vi "PicoScope5000aExampleAdvancedTriggerV2.vi"() -> ()   [LabVIEW 2010]
doc: "This example demonstrates how to use the PicoScope Labview library to collect data using Advanced triggers in block mode."
uses:
  shared/PicoBuffers.ctl
  <vilib>/Waveform/DWDTOps.llb/DWDT Analog to Digital.vi
  PicoScope5000aLib/PicoScope5000aDigitalChannelSettings.ctl
  PicoScope5000aLib/PicoScope5000aAnalogChannelSettings.ctl
  shared/Buffer and Transfer Settings.ctl
  shared/Acquisition Settings.ctl
panel:
  in  "Write to TDMS":bool
  in  "roundFaster":bool=TRUE
  in  "timeIntervalRequested":dbl min=0.0 format="%#6_6p"
  in  "Pulse Width Qualifier Settings":T1={"Direction"=2, "Lower Limit"=0, "Upper Limit"=0, "Pulse Width Type"=0} {"Pulse Width Type" items=["None", "Less Than", "Greater Than", "In Range", "Out of Range"]; "Direction" items=["Rising"=2, "Falling"=3, "Rising Lower"=7, "Above"=0, "Below"=1, "Rising or Falling"=4, "Falling Lower"=8, "Below Lower"=6, "Above Lower"=5]}
  in  "Trigger Conditions":T2={"Channel A"=1, "Channel B"=0, "Channel C"=0, "Channel D"=0, "Ext"=0, "Aux"=0, "PWQ"=0, "Digital Port 0"=0, "Digital Port 1"=0, "Condition Logic"=0} {"Digital Port 1" items=["Don't Care", "True", "False"]; "Digital Port 0" items=["Don't Care", "True", "False"]; "PWQ" items=["Don't Care", "True", "False"]; "Aux" items=["Don't Care", "True", "False"]; "Ext" items=["Don't Care", "True", "False"]; "Channel D" items=["Don't Care", "True", "False"]; "Channel C" items=["Don't Care", "True", "False"]; "Channel B" items=["Don't Care", "True", "False"]; "Channel A" items=["Don't Care", "True", "False"]; "Condition Logic" items=["AND", "OR", "XOR"]}
  in  "Pulse Width Qualifier Conditions":T3 {"Condition Logic" items=["AND", "OR", "XOR"]}
  in  "Digital Port  0":T4 {"Direction Channel 7" items=["Don't Care", "Low", "High", "Rising", "Falling"]; "Direction Channel 6" items=["Don't Care", "Low", "High", "Rising", "Falling"]; "Direction Channel 5" items=["Don't Care", "Low", "High", "Rising", "Falling"]; "Direction Channel 4" items=["Don't Care", "Low", "High", "Rising", "Falling"]; "Direction Channel 3" items=["Don't Care", "Low", "High", "Rising", "Falling"]; "Direction Channel 2" items=["Don't Care", "Low", "High", "Rising", "Falling"]; "Direction Channel 1" items=["Don't Care", "Low", "High", "Rising", "Falling"]; "Direction Channel 0" items=["Don't Care", "Low", "High", "Rising", "Falling"]}
  in  "Channel A Trigger Properties":T5={"thresholdUpper"=0, "thresholdUpperHysteresis"=0, "thresholdLower"=0, "thresholdLowerHysteresis"=0, "Threshold Mode"=0, "Direction"=2, "Available"=TRUE} {"Direction" items=["Above / Inside", "Below / Outside", "Rising / Enter", "Falling / Exit", "Rising or Falling / Enter or Exit", "Above Lower", "Below Lower", "Rising Lower", "Falling Lower", "Positive Runt", "Negative Runt"]; "Threshold Mode" items=["Level", "Window"]}
  out "overflow":i16 format="%010b"
  in  "Apply Settings":bool
  in  "Port 0 Settings":T6={"Enabled"=FALSE, "Logic Level"=9830} {"Logic Level" items=["1.5V TTL"=9830, "2.5V CMOS"=16383]}
  in  "Channel A Settings":T7={"Enabled"=TRUE, "Coupling"=1, "Range"=6, "Analogue Offset"=0.0, "Bandwidth Limit"=0} {"Bandwidth Limit" items=["Full", "20MHz"]; "Range" items=["10 mV", "20 mV", "50 mV", "100 mV", "200 mV", "500 mV", "1 V", "2 V", "5 V", "10 V", "20 V"]; "Coupling" items=["AC", "DC"]}
  out "USB 3.0 device on non-USB 3.0 Port":bool=TRUE
  out "USB Powered":bool=TRUE
  out "Device Info":T8={"Driver Version"="2.1.104.3324", "USB Version"="2.0", "Hardware"="1", "Variant"="5244A", "Batch and Serial"="CQ178/007", "Cal Date"="11Jun13", "Kernel Version"="1.0", "Digital HW Version"="1", "Analogue HW Version"="1", "MSO"=FALSE, "Number of channels"=2}
  out "error out":errorcluster
  in  "Data file":path=path "PicoScope5000aExampleBlock Data"
  in  "Buffer and Transfer Settings":T9={"startIndex"=0, "Samples"=5000000, "Down Sample Ratio"=1, "Down-Sample Mode"=0} {"Down-Sample Mode" items=["RAW none"=2147483648, "None"=0, "Aggregate"=1, "Decimate"=2, "Average"=4]; "Down Sample Ratio" step=1; "Samples" format="%_6p"}
  in  "Acquisition Settings":T10={"preTriggerSamples"=0, "postTriggerSamples"=5000000, "timebase"=0} {"postTriggerSamples" format="%_6p"; "preTriggerSamples" format="%_6p"}
  out "Properties Panel":T11 {"Max Total Capture Time Available (sec)" format="%.3p"; "Sample Frequency" format="%.6p"; "Sample Rate" format="%.3p"; "Max Samples Available" format="%_6p"; "Total Capture Time (sec)" format="%.3p"}
  out "Port 0":digitalwaveform(graph)={"t0"=timestamp(0 s since 1904-01-01), "dt"=8e-09, "Y"={"transitions"=[], "data"=[]}}
  in  "stop":bool
  out "Analog Channels":cluster{i32, sgl, "Data":dbl[]}[](graph)
  in  "Resolution":u32(ring) items=["8-bit"=0, "12-bit"=1, "14-bit"=2, "15-bit"=3, "16-bit"=4, "10-bit"=10]
  in  "Serial Number":string
  in  "Use Serial Number":bool
  in  "error in (no error)":errorcluster
  # "Bit 0 = ChA"
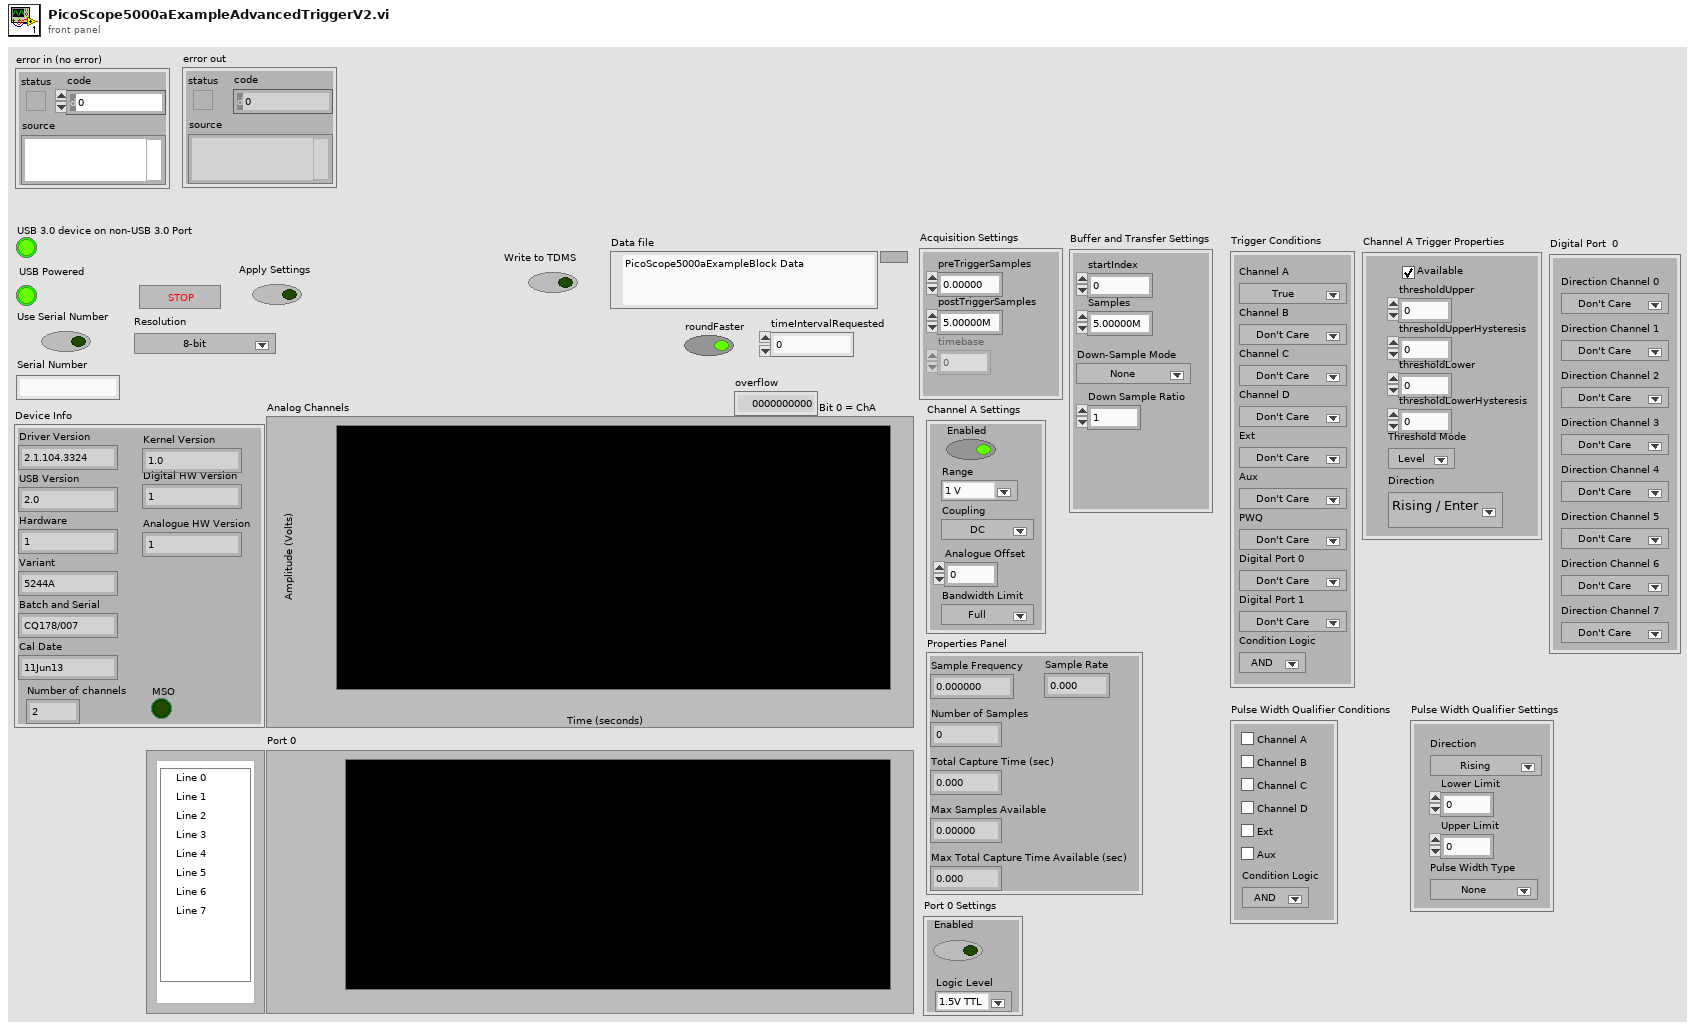
[diagram p1: front panel]
types:
  T1 = cluster{"Direction":u32, "Lower Limit":u32, "Upper Limit":u32, "Pulse Width Type":u32}
  T2 = cluster{"Channel A":u16, "Channel B":u16, "Channel C":u16, "Channel D":u16, "Ext":u16, "Aux":u16, "PWQ":u16, "Digital Port 0":u16, "Digital Port 1":u16, "Condition Logic":u16}
  T3 = cluster{"Channel A":bool, "Channel B":bool, "Channel C":bool, "Channel D":bool, "Aux":bool, "Condition Logic":u16, "Ext":bool}
  T4 = cluster{"Direction Channel 0":u16, "Direction Channel 1":u16, "Direction Channel 2":u16, "Direction Channel 3":u16, "Direction Channel 4":u16, "Direction Channel 5":u16, "Direction Channel 6":u16, "Direction Channel 7":u16}
  T5 = cluster{"thresholdUpper":i16, "thresholdUpperHysteresis":u16, "thresholdLower":i16, "thresholdLowerHysteresis":u16, "Threshold Mode":i32, "Direction":i32, "Available":bool}
  T6 = typedef "PicoScope5000aDigitalChannelSettings.ctl" = cluster{"Enabled":bool, "Logic Level":i16}
  T7 = typedef "PicoScope5000aAnalogChannelSettings.ctl" = cluster{"Enabled":bool, "Coupling":i16, "Range":u16, "Analogue Offset":sgl, "Bandwidth Limit":u32}
  T8 = cluster{"Driver Version":string, "USB Version":string, "Hardware":string, "Variant":string, "Batch and Serial":string, "Cal Date":string, "Kernel Version":string, "Digital HW Version":string, "Analogue HW Version":string, "MSO":bool, "Number of channels":i16}
  T9 = typedef "Buffer and Transfer Settings.ctl" = cluster{"startIndex":u64, "Samples":u64, "Down Sample Ratio":u64, "Down-Sample Mode":u32}
  T10 = typedef "Acquisition Settings.ctl" = cluster{"preTriggerSamples":u64, "postTriggerSamples":u64, "timebase":u32}
  T11 = cluster{"Sample Frequency":dbl, "Sample Rate":dbl, "Max Samples Available":u64, "Number of Samples":u64, "Total Capture Time (sec) ":dbl, "Max Total Capture Time Available (sec)":dbl}
  T12 = typedef "PicoBuffers.ctl" = cluster{"Max Buffer Pointers":u64[][][], "Min Buffer Pointers":u64[][][], "StreamingDataInfo":cluster{"Channel":u32, "Down-Sample Mode":u32, "PICO_DATA_TYPE":enum32{"PICO_INT8_T", "PICO_INT16_T", "PICO_INT32_T", "PICO_UINT32_T", "PICO_INT64_T", ""}, "Samples":i32, "bufferIndex":u64, "startIndex":i32, "overflow":i16}[][]}
  T13 = enum16{"open", "open or create", "create or replace", "create", "open (read-only)"}
  T14 = cluster{"Sample Frequency":sgl, "Sample Rate":sgl, "Max Samples Available":i32, "Number of Samples":u32, "Total Capture Time (sec) ":sgl, "Max Total Capture Time Available (sec)":sgl}
  T15 = cluster{"Channel A Buffer":i16[], "Channel B Buffer":i16[], "Channel C Buffer":i16[], "Channel D Buffer":i16[], "Channel E Buffer":i16[], "Channel F Buffer":i16[], "Channel G Buffer":i16[], "Channel H Buffer":i16[], "Port 0 Buffer":i16[], "Port 1 Buffer":i16[]}[]
  T16 = cluster{"Channel A Buffer":i16[], "Channel B Buffer":i16[], "Channel C Buffer":i16[], "Channel D Buffer":i16[], "Channel E Buffer":i16[], "Channel F Buffer":i16[], "Channel G Buffer":i16[], "Channel H Buffer":i16[], "Port 0 Buffer":i16[], "Port 1 Buffer":i16[]}
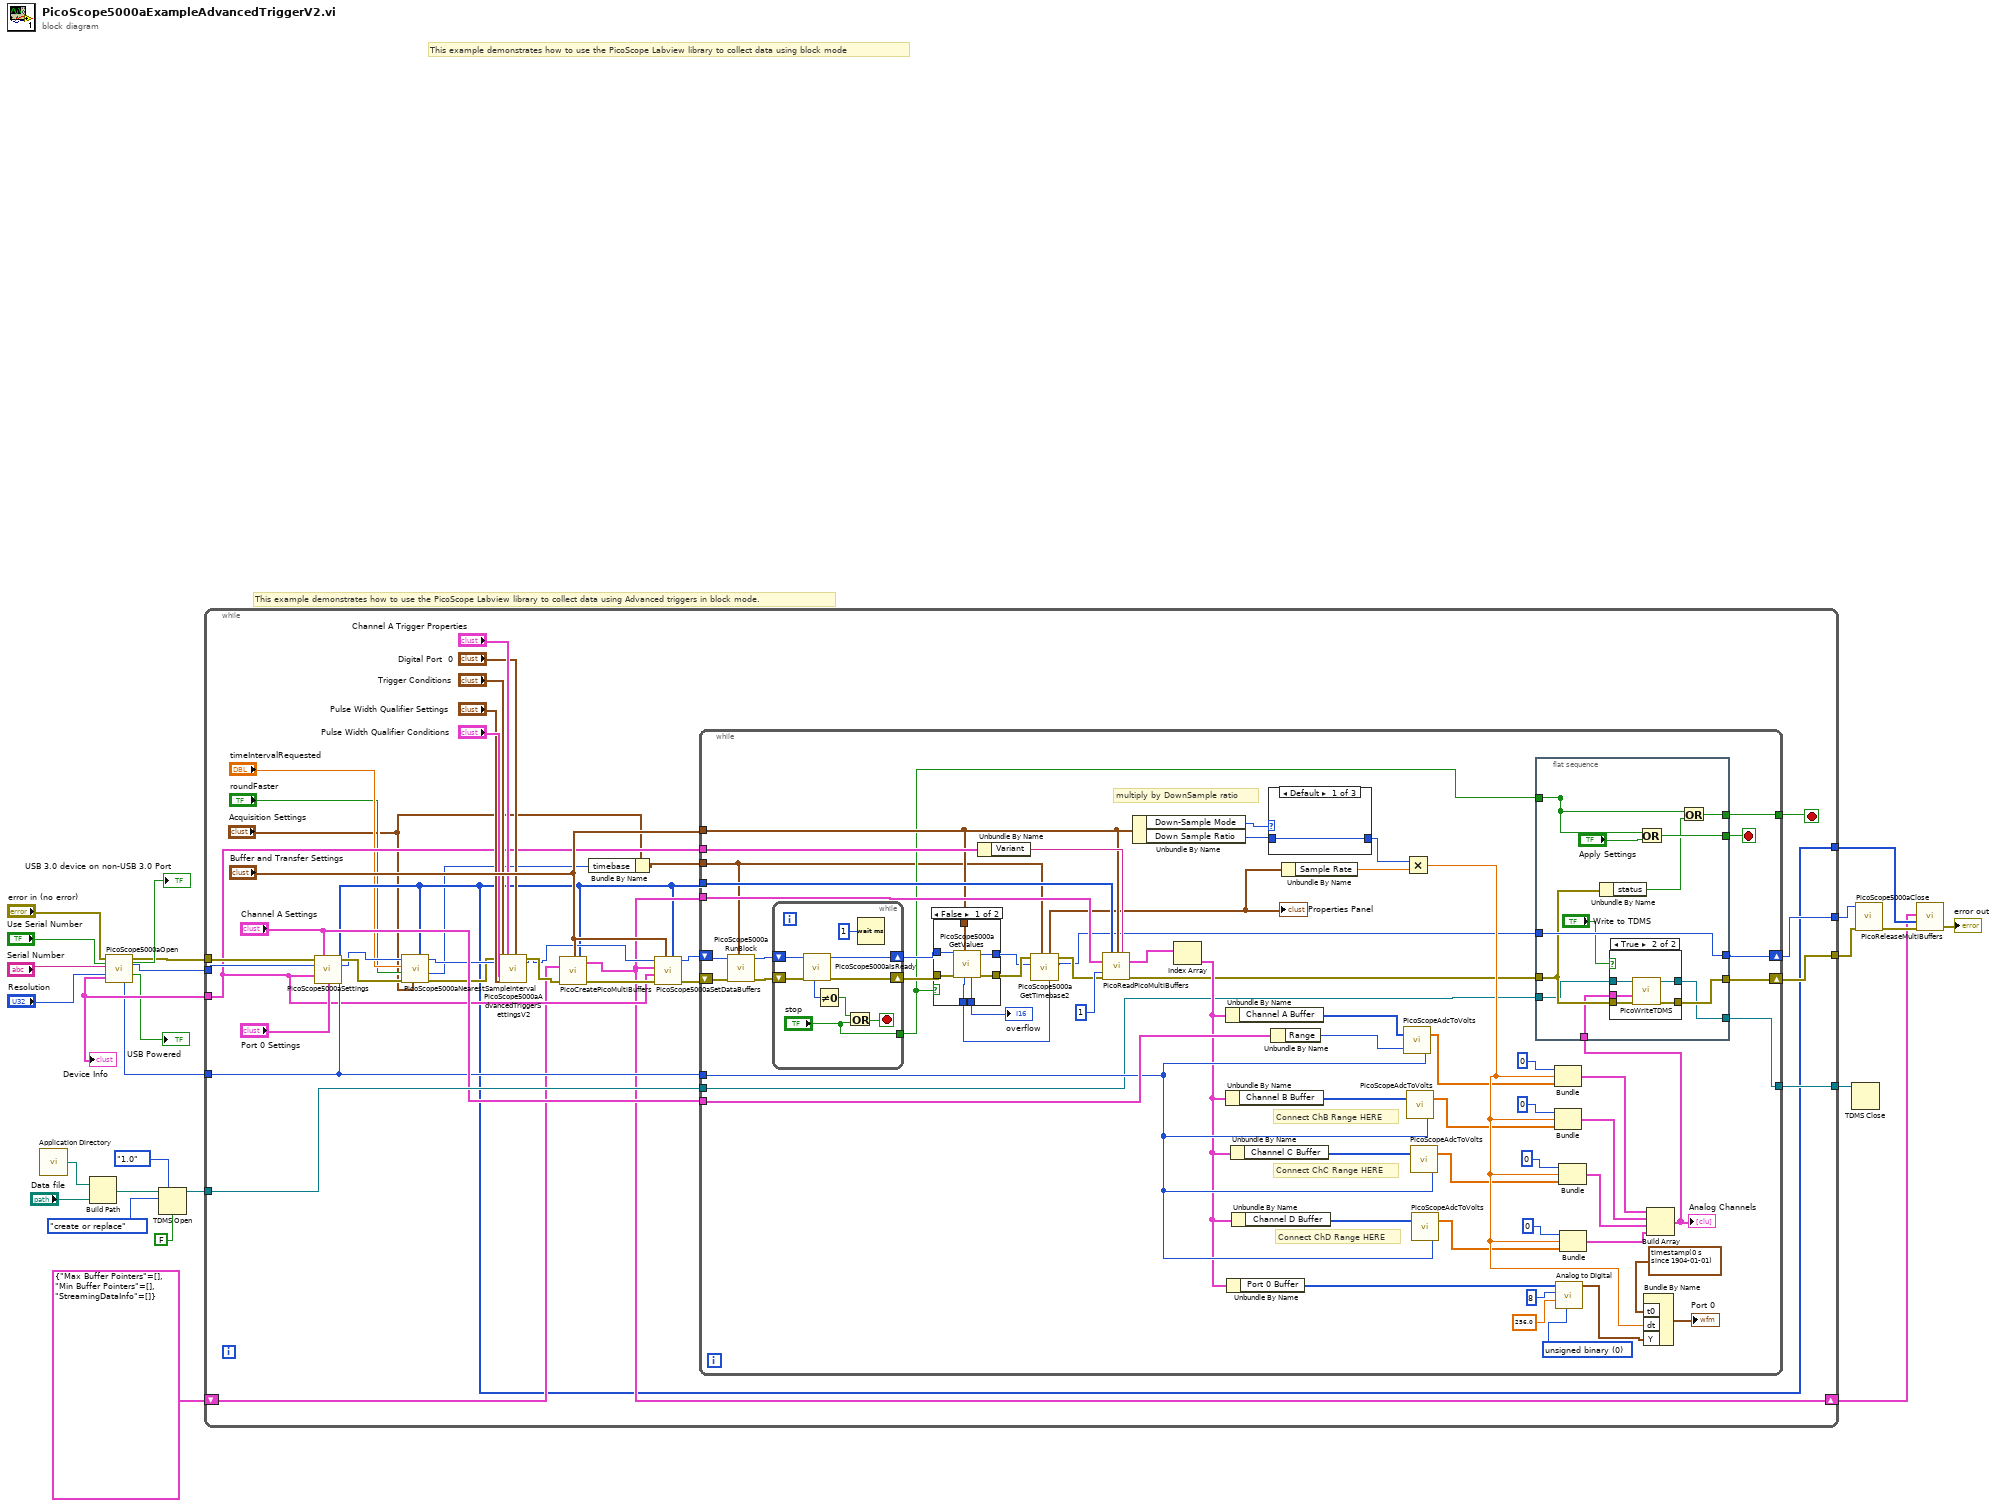
[diagram p0: block diagram]
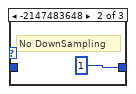
[diagram p4: hidden frame]
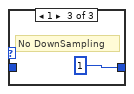
[diagram p5: hidden frame]
diagram:
  # "This example demonstrates how to use the PicoScope Labview library to collect data using Advanced triggers in block mode."
  # "This example demonstrates how to use the PicoScope Labview library to collect data using block mode"
  n1 = call <vilib>:"Application Directory.vi"() -> ("Application Directory"=w18:path)
  n2 = Build Path(base path=w18, name or relative path="Data file") -> (appended path=w19:path)
  n3 = call "PicoScope5000aOpen.vi"("error in (no error)"="error in (no error)", "Serial Number"="Serial Number", "Use Serial Number"="Use Serial Number", "Resolution"="Resolution") -> ("USB 3.0 device on non-USB 3.0 Port"=→"USB 3.0 device on non-USB 3.0 Port":bool, "error out"=w6:errorcluster, "handle"=w25:i16, "USB Powered"=→"USB Powered":bool, "Device Info"=w10:T8, "Max ADC value"=w9:i16)  [unwired: 6 in]
  "Device Info" <- w10
  n4 = TDMS Open(6:FALSE ("disable buffering? (T)"), 7:enum16{"1.0", "2.0"}."1.0" ("file format version (2.0)"), 10:T13."create or replace" ("operation (0:open)"), 11:w19) -> (3:w16:refnum<k34>)  [unwired: 2 in, 1 out]
  n5 = while {
    tunnel: w25 -> [w57]
    tunnel: w9 -> [w53]
    tunnel: [w31] -> w24
    tunnel: [w51] -> w17
    tunnel: w16 -> [w58]
    tunnel: w10 -> [w38]
    tunnel: w6 -> [w56]
    tunnel: [w52] -> w4
    tunnel: [w49] -> w5
    shift-right: [w36] -> w1
    shift-left: T12 {"Max Buffer Pointers"=[], "Min Buffer Pointers"=[], "StreamingDataInfo"=[]} ("Data Pointers") -> [w37]
    stop <- w50 stop-if-true
    n6 = call "PicoScope5000aSettings.vi"("error in"=w56, "Channel A Settings"="Channel A Settings", "Port 0 Settings"="Port 0 Settings", "handle in"=w57, "Device Info"=w38, "Max ADC value"=w53) -> ("error out"=w35:errorcluster, "handle out"=w34:i16, "enabled array"=w31:i16[])  [unwired: 7 in]
    n7 = call "PicoScope5000aNearestSampleInterval.vi"("Enabled array"=w31, "Acquisition Settings"="Acquisition Settings", "error in (no error)"=w35, "roundFaster"="roundFaster", "timeIntervalRequested"="timeIntervalRequested", "handle in"=w34) -> ("error out"=w32:errorcluster, "timebase"=w27:u32, "handle out"=w33:i16)  [unwired: 2 in, 1 out]
    n8 = call "PicoScope5000aAdvancedTriggerSettingsV2.vi"("error in"=w32, "handle in"=w33, "Trigger Conditions"="Trigger Conditions", "Channel A Trigger Properties"="Channel A Trigger Properties", "Digital Port  0"="Digital Port  0", "Pulse Width Qualifier Conditions"="Pulse Width Qualifier Conditions", "Pulse Width Qualifier Settings"="Pulse Width Qualifier Settings") -> ("error out"=w45:errorcluster, "handle out"=w44:i16)  [unwired: 11 in]
    n9 = call "PicoCreatePicoMultiBuffers.vi"("Buffer and Transfer Settings"="Buffer and Transfer Settings", "enabled array"=w31, "Data Pointers In"=w37, "error in (no error)"=w45) -> ("Data Pointers"=w36:T12, "error out"=w59:errorcluster)  [unwired: 10 in]
    n10 = Bundle By Name(cluster="Acquisition Settings", "timebase"=w27) -> (w28:T10)
    n11 = call "PicoScope5000aSetDataBuffers.vi"("enabled array"=w31, "Buffer and Transfer Settings"="Buffer and Transfer Settings", "error in (no error)"=w59, "Device Info"=w38, "Data Pointers In"=w36, "handle in"=w44) -> ("error out"=w48:errorcluster, "handle out"=w47:i16)  [unwired: 4 in]
    n12 = while {
      tunnel: w36 -> [w121]
      tunnel: "Buffer and Transfer Settings" -> [w72]
      tunnel: w31 -> [w113]
      tunnel: "Channel A Settings" -> [w112]
      tunnel: w28 -> [w63]
      tunnel: w53 -> [w111]
      tunnel: w38 -> [w108]
      tunnel: [w79] -> w50
      shift-right: [w81] -> w52
      shift-left: w48 -> [w73]
      shift-right: [w77] -> w49
      shift-left: w47 -> [w74]
      tunnel: w58 -> [w62]
      tunnel: [w60] -> w51
      stop <- w78 stop-if-true
      w98 = u16 0 items=["unsigned binary", "offset binary", "2's complement"] ("data format (offset binary)")
      # "Connect ChB Range HERE"
      # "Connect ChD Range HERE"
      # "Connect ChC Range HERE"
      # "multiply by DownSample ratio"
      n13 = call "PicoScope5000aRunBlock.vi"("Acquisition Settings"=w63, "error in (no error)"=w73, "handle in"=w74) -> ("error out"=w115:errorcluster, "handle out"=w114:i16)  [unwired: 5 in, 2 out]
      n14 = while {
        shift-right: [w157] -> w75
        shift-left: w115 -> [w158]
        shift-right: [w156] -> w76
        shift-left: w114 -> [w155]
        tunnel: ["stop"] -> w71
        stop <- w152 stop-if-true
        n15 = call "PicoScope5000aIsReady.vi"("error in (no error)"=w158, "handle in"=w155) -> ("error out"=w157:errorcluster, "handle out"=w156:i16, "ready"=w154:i16)  [unwired: 7 in]
        n16 = Not Equal To 0?(x=w154) -> (x != 0?=w153:bool)
        n17 = Or(x=w153, y="stop") -> (x .or. y?=w152:bool)
        n18 = Wait (ms)(milliseconds to wait=u32 1) -> ()  [unwired: 1 out]
      }
      n19 = case shown="False" w71 {
        tunnel: w75 -> [w128 w129]
        tunnel: w76 -> [w127 w130]
        tunnel: [w126 w130] -> w68
        tunnel: [w125 w129] -> w69
        tunnel: w72 -> [w124 _]
        tunnel: [w123 _] -> w70
        tunnel: [w122 _] -> w65
        frame False {
          n20 = call "PicoScope5000aGetValues.vi"("Buffer and Transfer Settings"=w124, "error in (no error)"=w128, "handle in"=w127) -> ("error out"=w125:errorcluster, "handle out"=w126:i16, "overflow"=w123:i16, "noOfSamples"=w122:u64)  [unwired: 5 in]
        }
        frame True {
        }
      }
      "overflow" <- w70
      n21 = Unbundle By Name(w108) -> ("Variant"=w109:string)
      n22 = call "PicoScope5000aGetTimebase2.vi"("Number of Samples"=w65, "Acquisition Settings"=w63, "handle in"=w68, "error in (no error)"=w69) -> ("handle out"=w66:i16, "error out"=w67:errorcluster, "Properties Panel"=w64:T14)  [unwired: 5 in]
      "Properties Panel" <- w64
      n23 = call "PicoReadPicoMultiBuffers.vi"("enabled array"=w113, "Buffer and Transfer Settings"=w72, "Variant"=w109, "Data Pointers"=w121, "No of Buffers"=1, "error in (no error)"=w67) -> ("MultiBuffers (Max or non-aggregated)"=w120:T15, "error out"=w80:errorcluster)  [unwired: 7 in, 1 out]
      n24 = Unbundle By Name(w72) -> ("Down-Sample Mode"=w118:u32, "Down Sample Ratio"=w119:u64)
      n25 = Index Array(array=w120) -> (element=w82:T16)  [unwired: 1 in]
      n26 = Unbundle By Name(w82) -> ("Channel A Buffer"=w91:i16[])
      n27 = Unbundle By Name(w82) -> ("Channel B Buffer"=w103:i16[])
      n28 = Unbundle By Name(w82) -> ("Port 0 Buffer"=w96:i16[])
      n29 = Unbundle By Name(w82) -> ("Channel C Buffer"=w89:i16[])
      n30 = Unbundle By Name(w82) -> ("Channel D Buffer"=w85:i16[])
      n31 = case shown="Default" w118 {
        tunnel: [w159 u64 1 ("Down Sample Ratio") u64 1 ("Down Sample Ratio")] -> w116
        tunnel: w119 -> [w159 _ _]
        frame Default {
        }
        frame -2147483648 {
          # "No DownSampling"
        }
        frame 1 {
          # "No DownSampling"
        }
      }
      n32 = Unbundle By Name(w112) -> ("Range"=w105:u16)
      n33 = Unbundle By Name(w64) -> ("Sample Rate"=w110:sgl)
      n34 = call "PicoScopeAdcToVolts.vi"("Max_adc"=w111, "Range Index"=w105, "Data"=w91) -> ("Data"=w92:dbl[])
      n35 = Multiply(x=w116, y=w110) -> (x*y=w117:sgl)
      n36 = call "PicoScopeAdcToVolts.vi"("Max_adc"=w111, "Data"=w103) -> ("Data"=w102:dbl[])  [unwired: 1 in]
      n37 = call "PicoScopeAdcToVolts.vi"("Max_adc"=w111, "Data"=w89) -> ("Data"=w88:dbl[])  [unwired: 1 in]
      n38 = call "PicoScopeAdcToVolts.vi"("Max_adc"=w111, "Data"=w85) -> ("Data"=w84:dbl[])  [unwired: 1 in]
      n39 = flat-sequence {
        tunnel: [w142] -> w78
        tunnel: [w137] -> _
        tunnel: [w139] -> w79
        tunnel: w66 -> [w138]
        tunnel: [w138] -> w77
        tunnel: w80 -> [w135]
        tunnel: [w136] -> w81
        tunnel: w71 -> [w137]
        tunnel: w62 -> [w134]
        tunnel: w61 -> [w132]
        tunnel: [w131] -> w60
        frame #0 {
          n40 = Unbundle By Name(w135) -> ("status"=w140:bool)
          n41 = case shown="True" "Write to TDMS" {
            tunnel: w135 -> [w143 w149]
            tunnel: [w143 w148] -> w136
            tunnel: w134 -> [w144 w147]
            tunnel: [w144 w146] -> w131
            tunnel: w132 -> [_ w145]
            frame False {
            }
            frame True {
              n42 = call "PicoWriteTDMS.vi"("error in (no error)"=w149, "Analog Channels"=w145, "Refnum in"=w147) -> ("error out"=w148:errorcluster, "Refnum out"=w146:refnum<k34>)  [unwired: 7 in]
            }
          }
          n43 = Or(x=w137, y="Apply Settings") -> (x .or. y?=w142:bool)
          n44 = Or(x=w137, y=w140) -> (x .or. y?=w139:bool)
        }
      }
      n45 = Bundle(0, w117, "Data"=w92) -> (w101:cluster{i32, sgl, "Data":dbl[]})  [unwired: 1 in]
      n46 = Bundle(0, w117, "Data"=w102) -> (w100:cluster{i32, sgl, "Data":dbl[]})  [unwired: 1 in]
      n47 = call-poly <vilib>:"Analog to Digital.vi"("data format (offset binary)"=w98, "full-scale range (pk-pk)"=256.0, "resolution (16 bit)"=8, "analog waveform"=w96) -> ("digital waveform"=w93:digitalwaveform)  [unwired: 4 in, 3 out]
      n48 = Bundle(0, w117, "Data"=w88) -> (w87:cluster{i32, sgl, "Data":dbl[]})  [unwired: 1 in]
      n49 = Bundle(0, w117, "Data"=w84) -> (w83:cluster{i32, sgl, "Data":dbl[]})  [unwired: 1 in]
      n50 = Bundle By Name("t0"=timestamp(0 s since 1904-01-01), "dt"=w117, "Y"=w93) -> (→"Port 0":digitalwaveform)  [unwired: 1 in]
      n51 = Build Array(w101, w100, w87, w83) -> (w61:cluster{i32, sgl, "Data":dbl[]}[])
      "Analog Channels" <- w61
    }
  }
  n52 = TDMS Close(11:w17) -> ()  [unwired: 1 in, 2 out]
  n53 = call "PicoScope5000aClose.vi"("error in (no error)"=w4, "handle in"=w5) -> ("error out"=w3:errorcluster)  [unwired: 8 in, 1 out]
  n54 = call "PicoReleaseMultiBuffers.vi"("error in (no error)"=w3, "Enabled array"=w24, "Data Pointers"=w1) -> ("error out"=→"error out":errorcluster)  [unwired: 7 in, 1 out]
